vi "RDC-Array-calc_propagation_const-measurement.vi"(5 "Short?":bool, 7 "dielectric":T1, 11 "Measured":T2) -> (2 "calc prop const":cdb[](array[numeric]))   [LabVIEW 2020, in "RDC-Reflection_Data_Computation.lvlib"]
doc: "Computes a propagation constant array from the reflection of the Measured Common Format cluster, using its unwrapped phase and RDC-coax-calculate_from_meas. Short? selects the short-circuit case."
uses:
  RDC-Reflection_Data_Computation.lvlib
  Reflector/RFH-common_data_format.ctl
  RDC-dielectric_types.ctl
  <vilib>/Analysis/NI_AALPro.lvlib
  Reflector/RFH-Reflection_File_Handler.lvlib
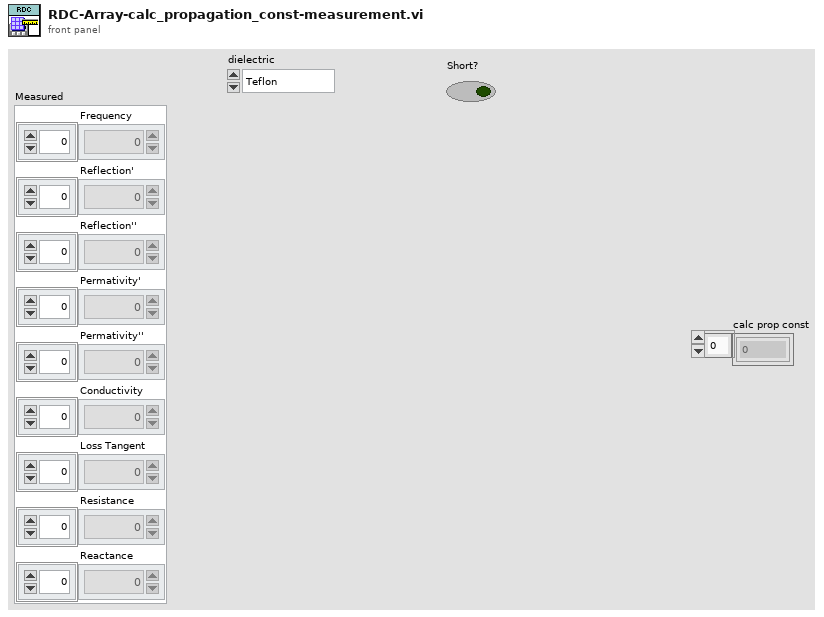
[diagram p1: front panel]
types:
  T1 = typedef "RDC-Reflection_Data_Computation.lvlib/RDC-dielectric_types.ctl" = enum16{"Teflon", "Eccostock 0005"}
  T2 = typedef "RFH-Reflection_File_Handler.lvlib/RFH-common_data_format.ctl" = cluster{"Frequency":dbl[], "Reflection'":dbl[], "Reflection''":dbl[], "Permativity'":dbl[], "Permativity''":dbl[], "Conductivity":dbl[], "Loss Tangent":dbl[], "Resistance":dbl[], "Reactance":dbl[]}
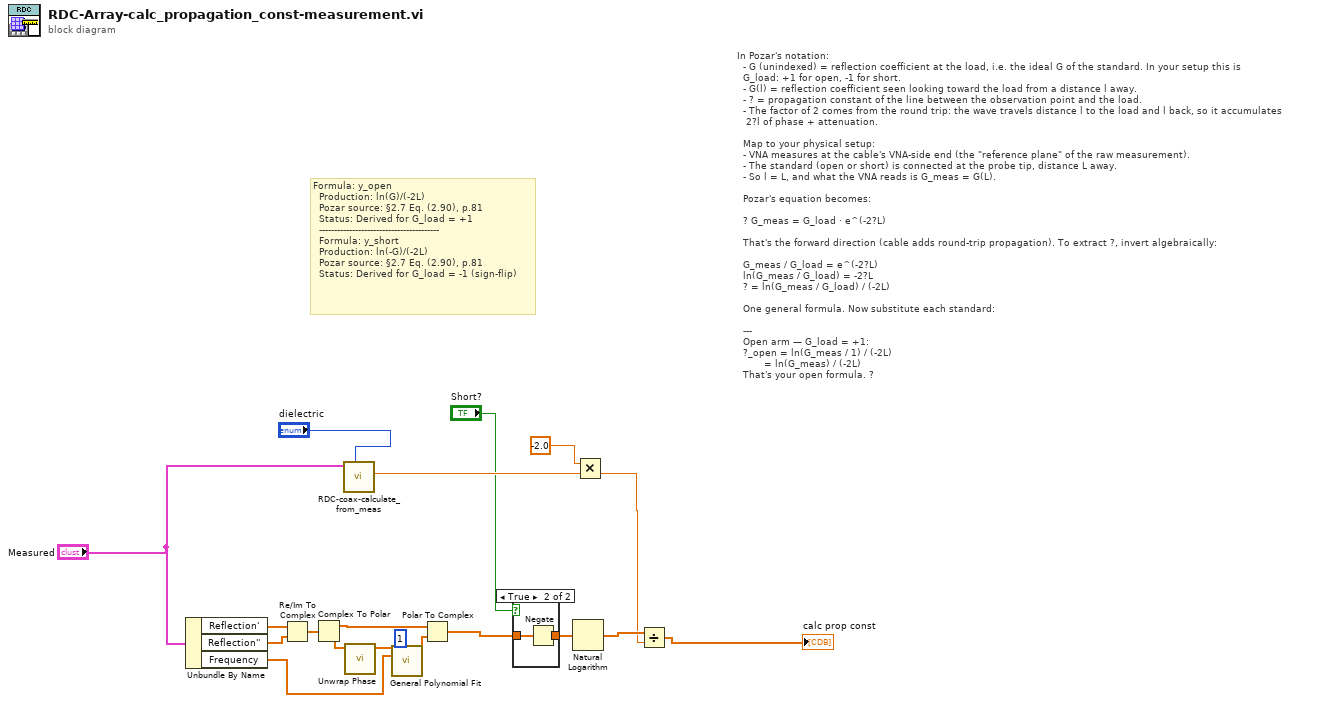
[diagram p0: block diagram]
diagram:
  # "In Pozar's notation:\n  - G (unindexed) = reflection coefficient at the load, i.e. the ideal G of the standard. In your setup this is\n  G_load: +1 for open, -1 for short.\n  - G(l) = reflection coefficient seen looking toward the load from a distance l away.\n  - ? = propagation constant of the line between the observation point and the load.\n  - The factor of 2 comes from the round trip: the wave travels distance l to the load and l back, so it accumulates\n   2?l of phase + attenuation.\n\n  Map to your physical setup:\n  - VNA measures at the cable's VNA-side end (the \"reference plane\" of the raw measurement).\n  - The standard (open or short) is connected at the probe tip, distance L away.\n  - So l = L, and what the VNA reads is G_meas = G(L).\n\n  Pozar's equation becomes:\n\n  ? G_meas = G_load · e^(-2?L)\n\n  That's the forward direction (cable adds round-trip propagation). To extract ?, invert algebraically:\n\n  G_meas / G_load = e^(-2?L)\n  ln(G_meas / G_load) = -2?L\n  ? = ln(G_meas / G_load) / (-2L)\n\n  One general formula. Now substitute each standard:\n\n  ---\n  Open arm — G_load = +1:\n  ?_open = ln(G_meas / 1) / (-2L)\n         = ln(G_meas) / (-2L)\n  That's your open formula. ?"
  # "Formula: y_open\n  Production: ln(G)/(-2L)\n  Pozar source: §2.7 Eq. (2.90), p.81\n  Status: Derived for G_load = +1\n  ----------------------------------------\n  Formula: y_short\n  Production: ln(-G)/(-2L)\n  Pozar source: §2.7 Eq. (2.90), p.81\n  Status: Derived for G_load = -1 (sign-flip)"
  n1 = Unbundle By Name("Measured") -> ("Reflection'"=w7:dbl[], "Reflection''"=w6:dbl[], "Frequency"=w5:dbl[])
  n2 = Re/Im To Complex(1:w6, 2:w7) -> (0:w15:cdb[])
  n3 = Complex To Polar(r * e^(i*theta)=w15) -> (r=w14:dbl[], theta=w9:dbl[])
  n4 = call "RDC-coax-calculate_from_meas.vi"("dielectric"="dielectric", "measurement"="Measured") -> ("lenght [m]"=w4:dbl)  [unwired: 7 in, 2 out]
  n5 = call <vilib>:"Unwrap Phase.vi"("Phase"=w9) -> ("Unwrapped Phase"=w11:dbl[])  [unwired: 9 in, 1 out]
  n6 = call <vilib>:"General Polynomial Fit.vi"("Y"=w11, "polynomial order"=1, "X"=w5) -> ("Best Polynomial Fit"=w8:dbl[])  [unwired: 9 in, 3 out]
  n7 = Polar To Complex(1:w8, 2:w14) -> (0:w13:cdb[])
  n8 = case shown="True" "Short?" {
    tunnel: [w20 w22] -> w17
    tunnel: w13 -> [w20 w21]
    frame False {
    }
    frame True {
      n9 = Negate(x=w21) -> (-x=w22:cdb[])
    }
  }
  n10 = Natural Logarithm(1:w17) -> (0:w16:cdb[])
  n11 = Multiply(x=-2.0, y=w4) -> (x*y=w2:dbl)
  n12 = Divide(x=w16, y=w2) -> (x/y=→"calc prop const":cdb[])
